vi "Own20261012_PublicDisconnectConnectorAll_v1.vi"() -> ()   [LabVIEW 2024]
panel:
  out "error out":errorcluster caption="错误输出"
  in  "target_path":path
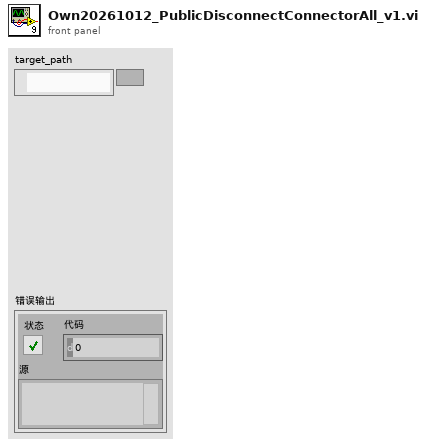
[diagram p1: front panel]
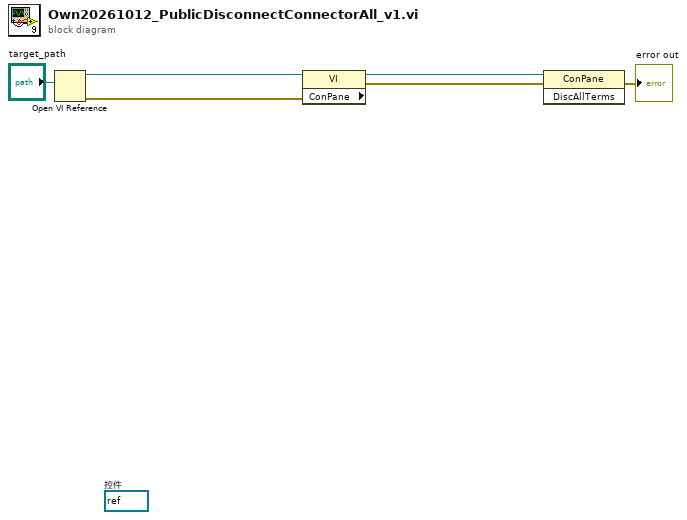
[diagram p0: block diagram]
diagram:
  (unwired) refnum<vi> refnum  # 控件
  n1 = Open VI Reference ("打开VI引用")(vi path="target_path") -> (vi reference=w5:refnum<vi>, error out=w2:errorcluster)  [unwired: 5 in]
  n2 = property on="属性节点" class="VI"(reference=w5, error in=w2) -> (error out=w1:errorcluster, "ConPane"=w4:refnum<vi>)  [unwired: 1 out]
  n3 = invoke class="ConPane" method="DiscAllTerms"(reference=w4, error in=w1) -> (error out=→"error out":errorcluster)  [unwired: 1 in, 2 out]
